vi "GetText.vi"(8 "error in":errorcluster, 11 "alarms module editor node in":refnum<class "alarms module editor node.lvclass">) -> (0 "error out":errorcluster, 1 "additional text":string, 2 "text":string, 3 "alarms module editor node out":refnum<class "alarms module editor node.lvclass">, 4 "glyph":string)   [LabVIEW 2013, in "alarms module editor node.lvclass"]
uses:
  alarms module editor node.lvclass
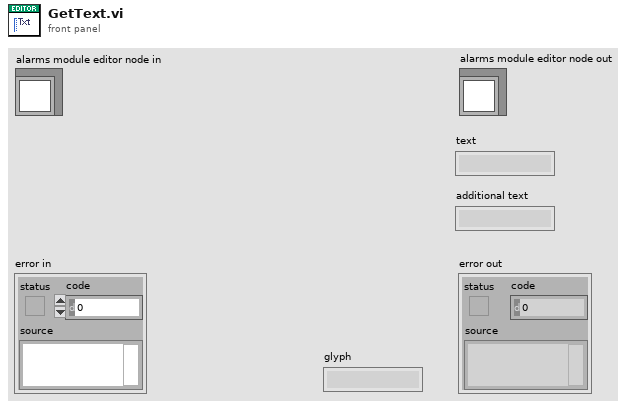
[diagram p1: front panel]
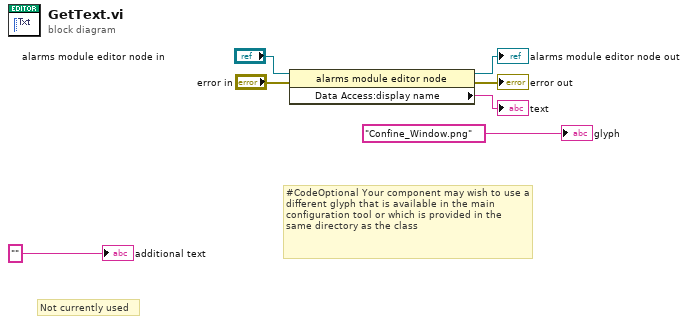
[diagram p0: block diagram]
diagram:
  # "Not currently used"
  # "#CodeOptional Your component may wish to use a different glyph that is available in the main configuration tool or which is provided in the same directory as the class"
  n1 = property class="alarms module editor node"(reference="alarms module editor node in", error in="error in") -> (reference out=→"alarms module editor node out":refnum<class "alarms module editor node.lvclass">, error out=→"error out":errorcluster, "Data Access:display name"=→"text":string)
  "additional text" <- "" ("additional text")
  "glyph" <- "Confine_Window.png" ("glyph")
